vi "SMTP Email Send Data.vi"(0 "recipients":string[](array[string]) caption="destinataires", 1 "mail server":string caption="serveur mail", 2 "return address":string caption="adresse de retour", 5 "subject ([No Subject])":string="[Sans objet]" caption="objet ([Sans objet])", 7 "message":string, 9 "data":string caption="données", 11 "error in (no error)":errorcluster caption="entrée d'erreur (pas d'erreur)", 12 "binary? (F)":bool caption="binaire ? (F)", 13 "MIME content-type (application/octet-stream)":string="application/octet-stream" caption="type de contenu MIME (application/octet-stream)") -> (4 "invalid recipients":string[](array[string]) caption="destinataires non valides", 15 "error out":errorcluster caption="sortie d'erreur")   [LabVIEW 2022 SP3, in "Copie de NI_SMTPEmail.lvlib"]
doc: "LabVIEW ne supporte plus ce VI. À la place, utilisez le VI Express Envoyer un e-mail.\n\nEnvoie un e-mail avec des données en pièce jointe à une liste de destinataires.\n\n<B>adresse de retour</B> est l'adresse-email de l'expéditeur du message. Si vous ne spécifiez pas d'adresse de retour, une chaîne vide est envoyée au serveur. Vous n'êtes pas obligé d'inclure une adresse de retour pour que ce VI fonctionne, mais certains serveurs de messagerie n'acceptent pas les messages si ces informations sont absentes. \n<B>serveur mail</B> est le nom ou l'adresse IP d'un serveur SMTP valide. Si vous passez une chaîne vide à cette entrée, LabVIEW n'accepte pas la connexion réseau et renvoie l'erreur 63. \n<B>destinataires</B> est le tableau de chaînes qui contient les adresses e-mail des destinataires du message. Chaque adresse peut être un élément de tableau séparé. \n<B>objet</B> est la ligne d'objet du message. La valeur par défaut est [Sans objet]. \n<B>message</B> correspond au message textuel de l'e-mail, formaté avec le jeu de caractères système. LabVIEW convertit cette chaîne en format UTF-8 avant d'envoyer l'e-mail. \n<B>données</B> contient les informations à joindre à l'e-mail, au format texte ou binaire. Si les données sont binaires, vous devez définir <B>binaire</B> à VRAI et définir aussi <B>type de contenu MIME</B>.\n<B>entrée d'erreur</B> décrit les conditions d'erreur survenues avant l'exécution de ce nœud. Cette entrée fournit la fonctionnalité d'entrée d'erreur standard. \n<B>binaire ?</B> spécifie si la pièce jointe est au format texte, décrite par le paramètre <B>jeu de caractères</B>, ou binaire, décrite par le paramètre <B>type de contenu MIME</B>. La valeur par défaut est FAUX, ce qui spécifie une pièce jointe de type texte.\n<B>type de contenu MIME</B> détermine le type de contenu pour une pièce jointe de type binaire. Vous pouvez spécifier n'importe quel type de contenu supporté par la norme RFC 2045, y compris les types de contenu courants suivants :\n\napplication/octet-stream (valeur par défaut) : indique un fichier binaire générique.\n\nimage/jpeg : indique des images JPEG.\n\ntext/html : indique des documents au format HTML.\n\n<B>destinataires non valides</B> liste les destinataires rejetés par le serveur mail. \n<B>sortie d'erreur</B> contient des informations sur l'erreur. Cette sortie fournit la fonctionnalité de sortie d'erreur standard."
uses:
  Copie de NI_SMTPEmail.lvlib
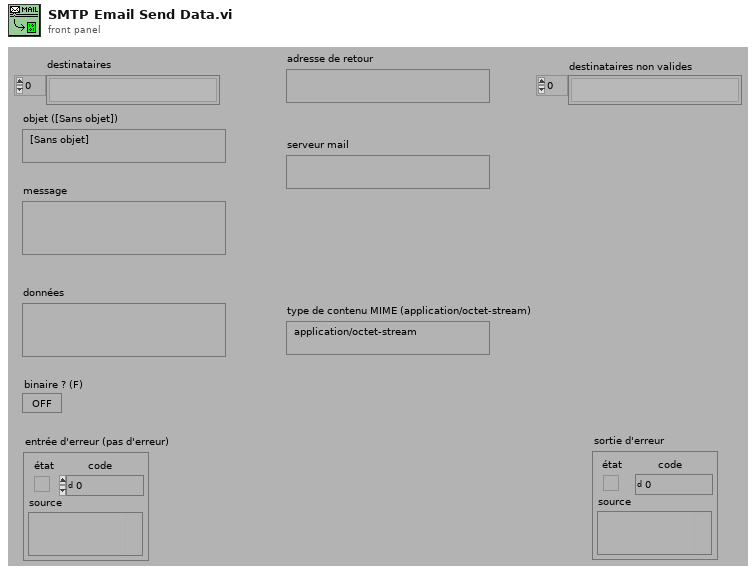
[diagram p1: front panel]
types:
  T1 = cluster{path, "data":string, "binary? (F)":bool, "MIME content-type (application/octet-stream)":string}
  T2 = cluster{path, "data":string, "binary? (F)":bool, "MIME content-type (application/octet-stream)":string}[]
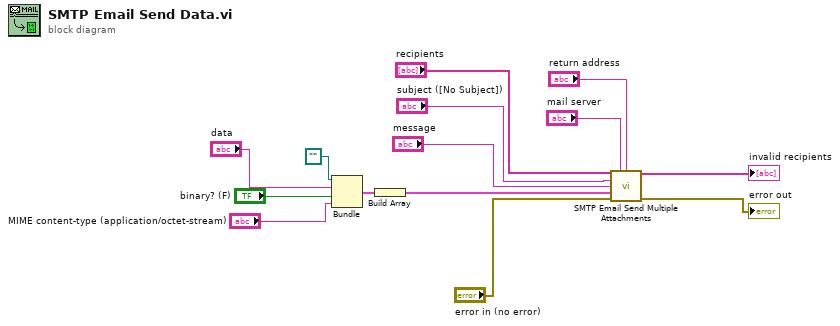
[diagram p0: block diagram]
diagram:
  n1 = Bundle(path "", "data"="data", "binary? (F)"="binary? (F)", "MIME content-type (application/octet-stream)"="MIME content-type (application/octet-stream)") -> (w3:T1)  [unwired: 1 in]
  n2 = Build Array(w3) -> (w2:T2)
  n3 = call "SMTP Email Send Multiple Attachments.vi"("recipients"="recipients", "mail server"="mail server", "return address"="return address", "subject ([No Subject])"="subject ([No Subject])", "message"="message", "attachments"=w2, "error in (no error)"="error in (no error)") -> ("invalid recipients"=→"invalid recipients":string[], "error out"=→"error out":errorcluster)  [unwired: 7 in]
